vi "error.vi"(8 "error in":errorcluster, 11 "REST Response":string) -> (0 "error out":errorcluster, 3 "Error Formatted Response":string)   [LabVIEW 2020, in "Nominal Client.lvclass"]
uses:
  Nominal Client.lvclass
  859f8e04-e495-489b-b5b4-7ac163f56130.vi
  <vilib>/JDP Science/JSONtext/JSON text to Variant.vi
  <vilib>/JDP Science/JSONtext/LVClass Serializer/JSONtext LVClass Serializer.lvclass
  Nominal Client.lvclass/Nominal Client.ctl
  <vilib>/JDP Science/JSONtext/JSONtext.lvlib
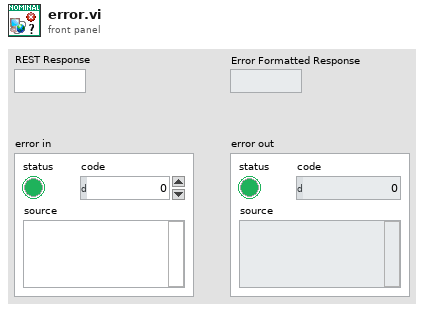
[diagram p1: front panel]
types:
  T1 = cluster{"errorCode":string, "errorName":string, "errorInstanceId":string}
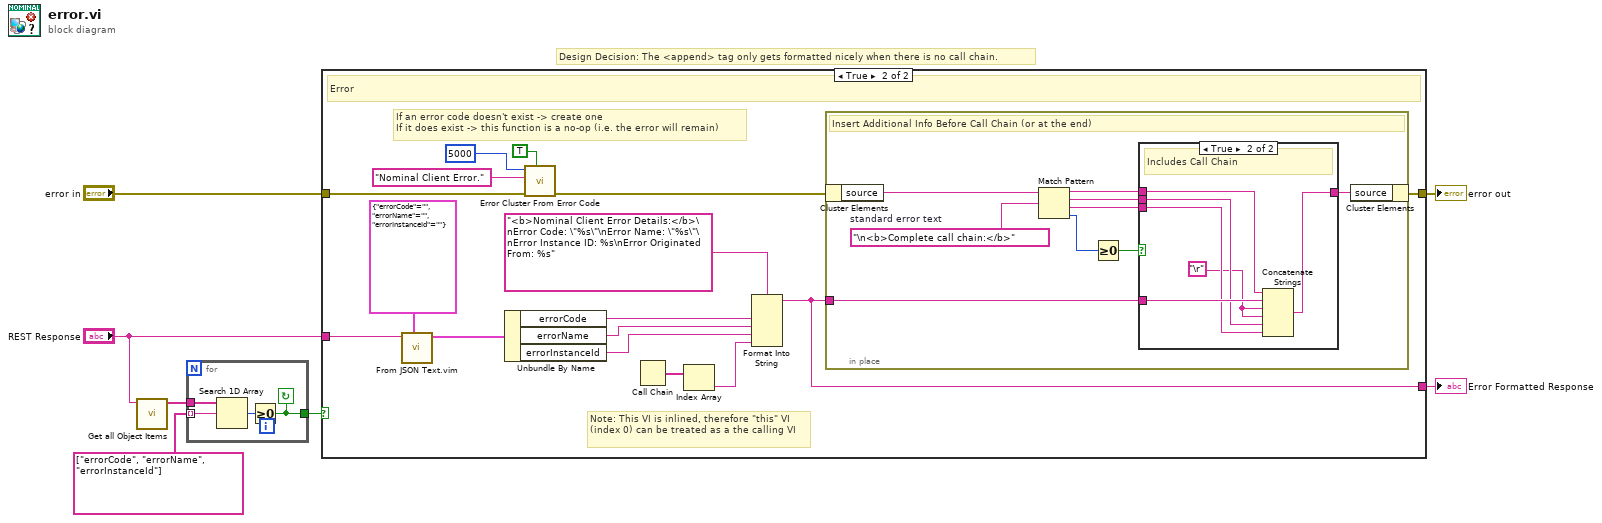
[diagram p0: block diagram]
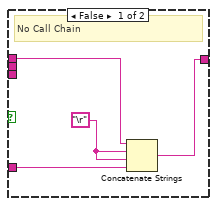
[diagram p3: hidden frame]
diagram:
  # "Design Decision: The <append> tag only gets formatted nicely when there is no call chain."
  n1 = call <vilib>:"Get all Object Items.vi"("JSON"="REST Response") -> ("Item Names"=w6:string[])  [unwired: 7 in, 3 out]
  n2 = for {
    tunnel: w6 -> [w11]
    tunnel: string[] ["errorCode", "errorName", "errorInstanceId"] ("Item Names") -> [w10] mode=indexing
    tunnel: [w8] -> w5
    stop <- w8 continue-if-true
    n3 = Search 1D Array(1D array=w11, element=w10) -> (index of element=w9:i32)  [unwired: 1 in]
    n4 = Greater Or Equal To 0?(x=w9) -> (x >= 0?=w8:bool)
  }
  n5 = case shown="True" w5 {
    tunnel: [w13 w27] -> w3
    tunnel: "REST Response" -> [w12 w20]
    tunnel: "error in" -> [w13 w16]
    tunnel: [w12 w14] -> w1
    frame False {
      # "Not an error"
    }
    frame True {
      # "If an error code doesn't exist -> create one\nIf it does exist -> this function is a no-op (i.e. the error will remain)"
      # "Note: This VI is inlined, therefore \"this\" VI (index 0) can be treated as a the calling VI"
      # "Error"
      n6 = call "From JSON Text.vim"("Data Type and Default Value"=T1 {"errorCode"="", "errorName"="", "errorInstanceId"=""}, "JSON"=w20) -> ("Data out"=w25:T1)  [unwired: 8 in, 1 out]
      n7 = Unbundle By Name(w25) -> ("errorCode"=w23:string, "errorName"=w22:string, "errorInstanceId"=w21:string)
      n8 = call <vilib>:"Error Cluster From Error Code.vi"("show call chain? (False)"=TRUE, "error in (no error)"=w16, "error message (\"\")"="Nominal Client Error." ("error message (\"\")"), "error code (0)"=5000) -> ("error out"=w17:errorcluster)  [unwired: 5 in]
      n9 = Call Chain() -> (call chain=w29:string[])
      n10 = Index Array(array=w29) -> (element=w24:string)  [unwired: 1 in]
      n11 = Format Into String(format string="<b>Nominal Client Error Details:</b>\nError Code: \"%s\"\nError Name: \"%s\"\nError Instance ID: %s\nError Originated From: %s" ("search string"), w23, w22, w21, w24) -> (resulting string=w14:string)  [unwired: 2 in, 1 out]
      n12 = in-place {
        in-place-border: w14 -> [w37]
        w35 = "\n<b>Complete call chain:</b>"  # standard error text
        # "Insert Additional Info Before Call Chain (or at the end)"
        n13 = in-place-cluster #1(w17) -> ("source"=w36:string)
        n14 = Match Pattern(string=w36, regular expression=w35) -> (before substring=w32:string, match substring=w33:string, after substring=w34:string, offset past match=w31:i32)  [unwired: 1 in]
        n15 = Greater Or Equal To 0?(x=w31) -> (x >= 0?=w30:bool)
        n16 = case shown="True" w30 {
          tunnel: [w41 w48] -> w38
          tunnel: w37 -> [w39 w47]
          tunnel: w34 -> [_ w46]
          tunnel: w33 -> [_ w45]
          tunnel: w32 -> [w42 w44]
          frame False {
            w40 = "\r"
            # "No Call Chain"
            n17 = Concatenate Strings(w42, w40, w40, w39) -> (w41:string)
          }
          frame True {
            w43 = "\r"
            # "Includes Call Chain"
            n18 = Concatenate Strings(w44, w47, w43, w43, w45, w46) -> (w48:string)
          }
        }
        n19 = in-place-cluster #1("source"=w38) -> (w27:errorcluster)
      }
    }
  }
  "error out" <- w3
  "Error Formatted Response" <- w1
